vi "WriteCoreLoop_v2.vi"(5 "InitialFiles Format":T1=enum."Binary Files", 7 "Controls ref.":T2, 8 "data error in":errorcluster, 9 "data queue in":refnum<queue>, 10 "control queue in":errorcluster, 11 "control queue in":refnum<queue>) -> (0 "error out":errorcluster)   [LabVIEW 2013]
uses:
  ControlDef/Files_Format.ctl
  ControlDef/ProcessingMode.ctl
  Signal_Segment.ctl
  SaveControlsRef.ctl
  WriterState.ctl
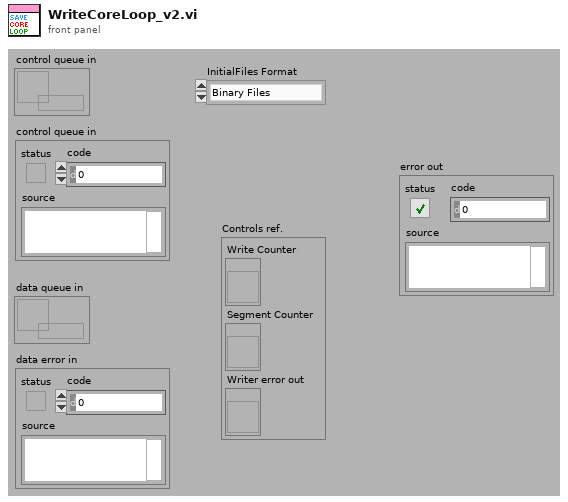
[diagram p1: front panel]
types:
  T1 = typedef "Files_Format.ctl" = enum16{"Text Files", "mzML Files", "Binary Files", "BioMap Files", "imzML Files"}
  T2 = typedef "SaveControlsRef.ctl" = cluster{"Write Counter":refnum<vi>, "Segment Counter":refnum<vi>, "Writer error out":refnum<vi>}
  T3 = typedef "WriterState.ctl" = cluster{"State":enum16{"Open", "Close", "ChangeFormat", "SetHeader", "QuitProg."}, "Params":variant}
  T4 = enum16{"Open", "Close", "ChangeFormat", "SetHeader", "QuitProg."}
  T5 = typedef "Signal_Segment.ctl" = cluster{"SampleRate":dbl, "TrigDelay":dbl, "SpecLength":dbl, "DAQ_Range":dbl, "Average#":i32, "Position":dbl[], "Spectrum":sgl[], "Calibr.":dbl[], "Pressure":dbl, "Desp_LaserEnergy":dbl, "PI_LaserEnergy":dbl, "Voltages Table":sgl[][], "ProcMode":T6, "Threshold":dbl, "Comment":string, "TickCount":dbl, "Time Stamp":timestamp}
  T6 = typedef "ProcessingMode.ctl" = enum16{"None", "Drop by Threshold", "TDC Simulate", "SetFilter"}
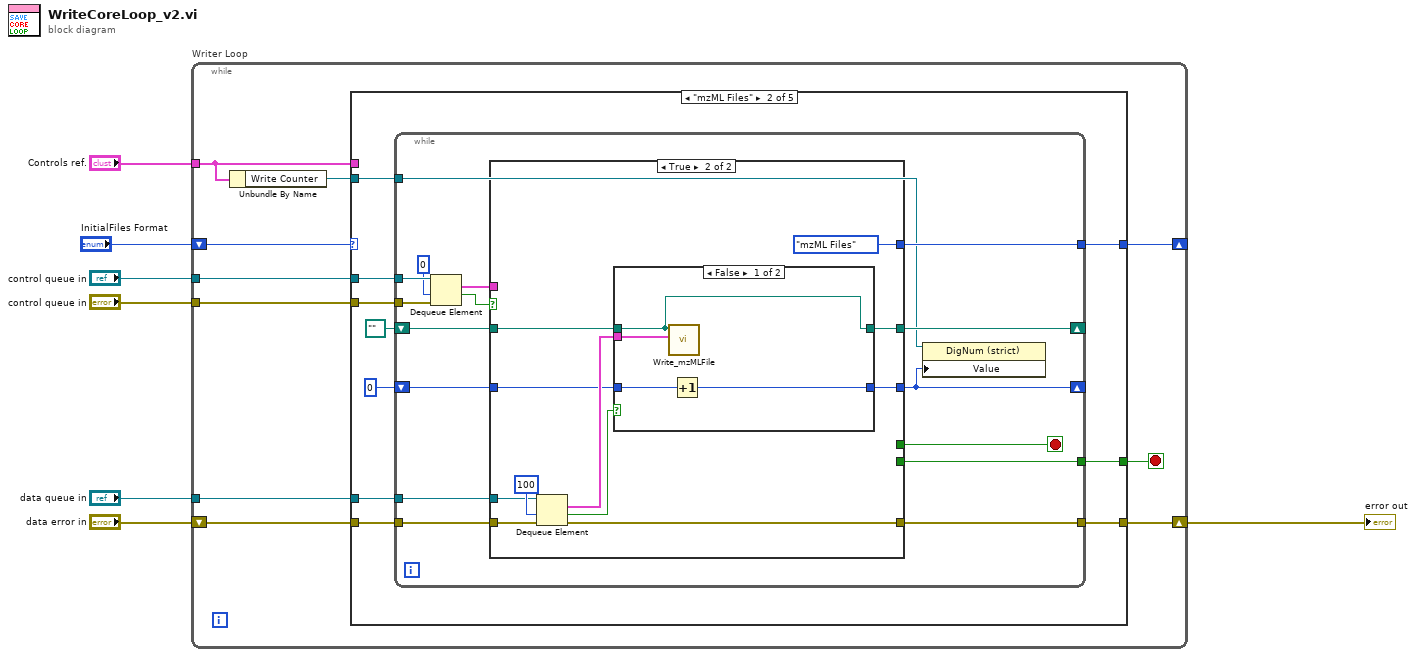
[diagram p0: block diagram]
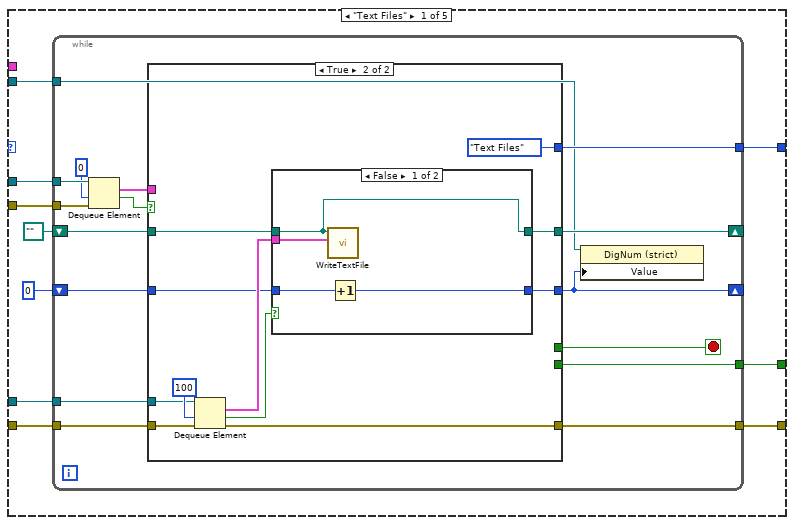
[diagram p2: hidden frame]
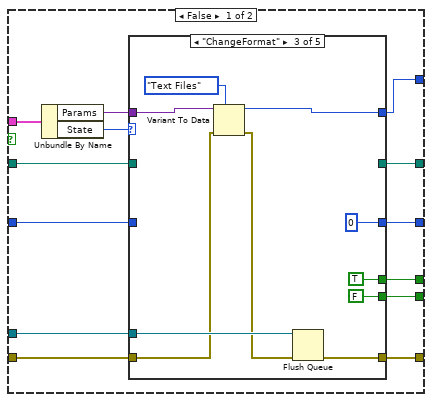
[diagram p3: hidden frame]
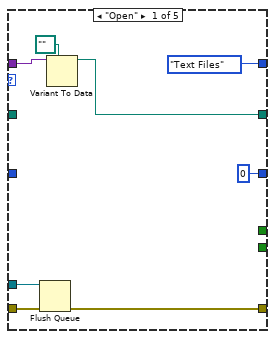
[diagram p4: hidden frame]
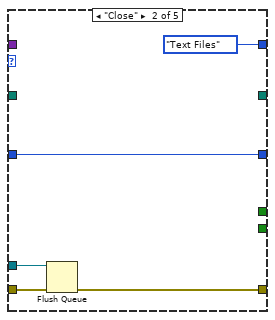
[diagram p5: hidden frame]
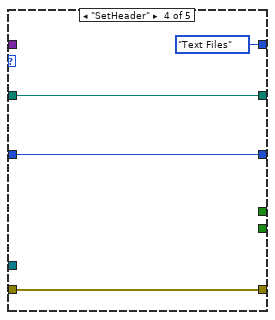
[diagram p6: hidden frame]
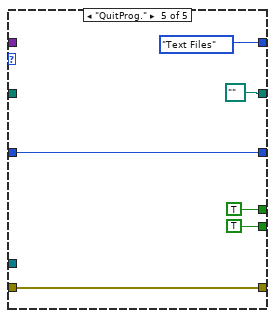
[diagram p7: hidden frame]
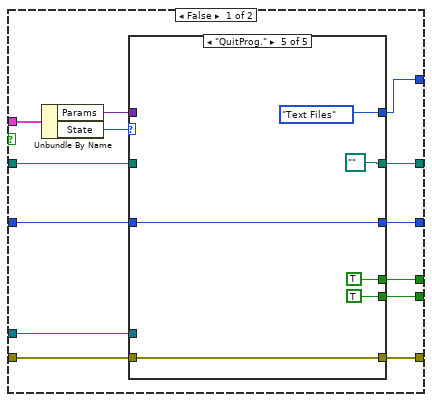
[diagram p9: hidden frame]
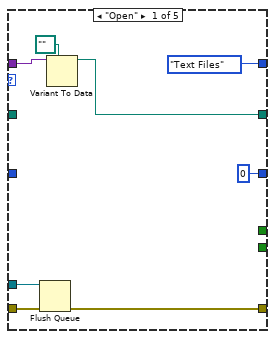
[diagram p10: hidden frame]
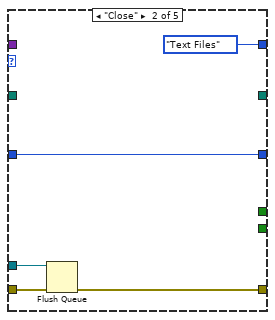
[diagram p11: hidden frame]
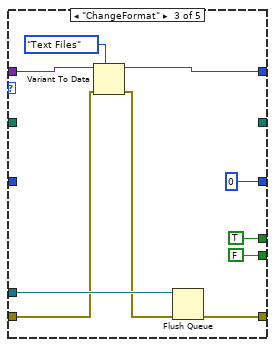
[diagram p12: hidden frame]
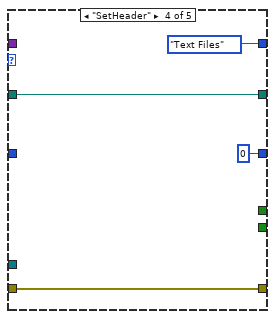
[diagram p13: hidden frame]
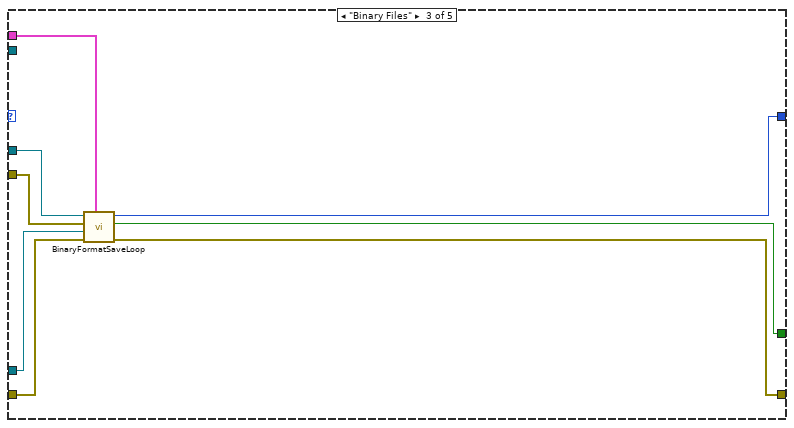
[diagram p15: hidden frame]
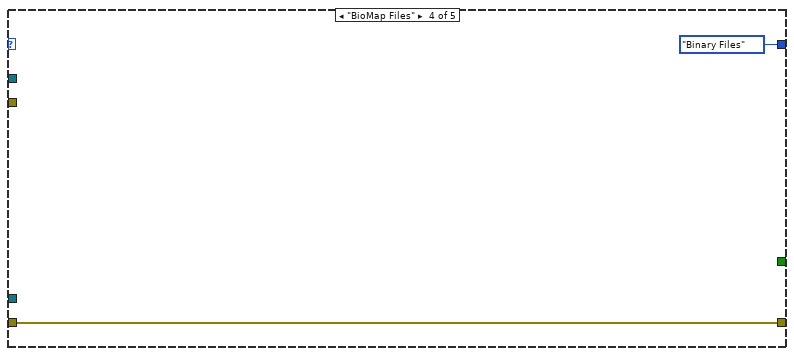
[diagram p16: hidden frame]
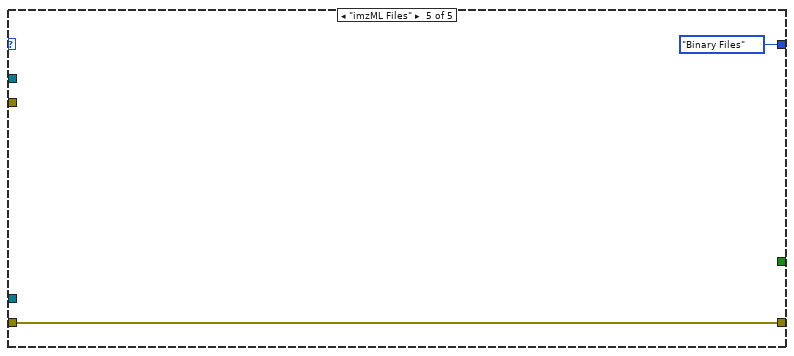
[diagram p17: hidden frame]
diagram:
  n1 = while "Writer Loop" {
    shift-right: [w10] -> w2
    shift-left: "data error in" -> [w15]
    tunnel: "data queue in" -> [w16]
    tunnel: "Controls ref." -> [w9]
    tunnel: "control queue in" -> [w14]
    tunnel: "control queue in" -> [w13]
    shift-right: [w11] -> _
    shift-left: "InitialFiles Format" -> [w12]
    stop <- w17 stop-if-true
    n2 = Unbundle By Name(w9) -> ("Write Counter"=w8:refnum<vi>)
    n3 = case shown="\"mzML Files\"" w12 {
      tunnel: [w27 w116 w203 _ _] -> w17
      tunnel: w16 -> [w25 w114 w202 _ _]
      tunnel: w15 -> [w24 w113 w201 w205 w207]
      tunnel: w14 -> [w23 w112 w200 _ _]
      tunnel: w13 -> [w22 w111 w199 _ _]
      tunnel: [w21 w110 w198 Files_Format."Binary Files" ("Format") Files_Format."Binary Files" ("Format")] -> w11
      tunnel: [w19 w108 w196 w205 w207] -> w10
      tunnel: w9 -> [_ _ w197 _ _]
      tunnel: w8 -> [w18 w107 _ _ _]
      frame "Text Files" {
        n4 = while {
          tunnel: [w41] -> w27
          shift-right: [w29] -> _
          shift-left: 0 -> [w43]
          tunnel: w25 -> [w36]
          tunnel: w24 -> [w35]
          shift-right: [w31] -> _
          shift-left: path "" ("file path") -> [w42]
          tunnel: w23 -> [w40]
          tunnel: w22 -> [w39]
          tunnel: [w32] -> w21
          tunnel: [w30] -> w19
          tunnel: w18 -> [w28]
          stop <- w33 stop-if-true
          n5 = Dequeue Element(queue=w40, timeout in ms (-1)=0, error in (no error)=w39) -> (element=w34:T3, timed out?=w37:bool)  [unwired: 2 out]
          n6 = case shown="True" w37 {
            tunnel: w43 -> [w50 w94]
            tunnel: w42 -> [w54 w96]
            tunnel: [w51 w93] -> w29
            tunnel: [w53 _] -> w41
            tunnel: w36 -> [w48 w99]
            tunnel: w35 -> [w47 w98]
            tunnel: w34 -> [w56 _]
            tunnel: [w52 _] -> w33
            tunnel: [w44 Files_Format."Text Files" ("Format")] -> w32
            tunnel: [w49 w91] -> w31
            tunnel: [w46 w90] -> w30
            frame False {
              n7 = Unbundle By Name(w56) -> ("Params"=w45:variant, "State"=w55:T4)
              n8 = case shown="\"ChangeFormat\"" w55 {
                tunnel: w54 -> [_ _ _ w81 _]
                tunnel: [w57 _ _ w81 path "" ("file path")] -> w49
                tunnel: [_ _ FALSE _ TRUE] -> w53
                tunnel: [_ _ TRUE _ TRUE] -> w52
                tunnel: [Files_Format."Text Files" ("Format") Files_Format."Text Files" ("Format") w73 Files_Format."Text Files" ("Format") Files_Format."Text Files" ("Format")] -> w44
                tunnel: [0 w69 0 w82 w87] -> w51
                tunnel: w50 -> [_ w69 _ w82 w87]
                tunnel: w48 -> [w61 w67 w76 _ _]
                tunnel: w47 -> [w62 w68 w71 w80 w84]
                tunnel: [w60 w66 w75 w80 w84] -> w46
                tunnel: w45 -> [w58 _ w74 _ _]
                frame "Open" {
                  n9 = Flush Queue(queue=w61, error in (no error)=w62) -> (error out=w60:errorcluster)  [unwired: 2 out]
                  n10 = Variant To Data(type=path "" ("path"), Variant=w58) -> (data=w57:path)  [unwired: 1 in, 1 out]
                }
                frame "Close" {
                  n11 = Flush Queue(queue=w67, error in (no error)=w68) -> (error out=w66:errorcluster)  [unwired: 2 out]
                }
                frame "ChangeFormat" {
                  n12 = Variant To Data(error in=w71, type=Files_Format."Text Files" ("Format"), Variant=w74) -> (data=w73:T1, error out=w72:errorcluster)
                  n13 = Flush Queue(queue=w76, error in (no error)=w72) -> (error out=w75:errorcluster)  [unwired: 2 out]
                }
                frame "SetHeader" {
                }
                frame "QuitProg." {
                }
              }
            }
            frame True {
              n14 = Dequeue Element(queue=w99, timeout in ms (-1)=100, error in (no error)=w98) -> (element=w97:T5, timed out?=w92:bool, error out=w90:errorcluster)  [unwired: 1 out]
              n15 = case shown="False" w92 {
                tunnel: w97 -> [w104 _]
                tunnel: w96 -> [w103 w106]
                tunnel: [w103 w106] -> w91
                tunnel: w94 -> [w102 w105]
                tunnel: [w101 w105] -> w93
                frame False {
                  n16 = call "WriteTextFile.vi"("Signal Segment"=w104, "Filename"=w103) -> ()  [unwired: 9 in, 1 out]
                  n17 = Increment(x=w102) -> (x+1=w101:i32)
                }
                frame True {
                }
              }
            }
          }
          n18 = property class="DigNum (strict)"(reference=w28, "Value"=w29) -> ()  [unwired: 1 in, 2 out]
        }
      }
      frame "mzML Files" {
        n19 = while {
          tunnel: [w130] -> w116
          shift-right: [w118] -> _
          shift-left: 0 -> [w132]
          tunnel: w114 -> [w125]
          tunnel: w113 -> [w124]
          shift-right: [w120] -> _
          shift-left: path "" ("file path") -> [w131]
          tunnel: w112 -> [w129]
          tunnel: w111 -> [w128]
          tunnel: [w121] -> w110
          tunnel: [w119] -> w108
          tunnel: w107 -> [w117]
          stop <- w122 stop-if-true
          n20 = Dequeue Element(queue=w129, timeout in ms (-1)=0, error in (no error)=w128) -> (element=w123:T3, timed out?=w126:bool)  [unwired: 2 out]
          n21 = case shown="True" w126 {
            tunnel: w132 -> [w139 w183]
            tunnel: w131 -> [w143 w185]
            tunnel: [w140 w182] -> w118
            tunnel: [w142 _] -> w130
            tunnel: w125 -> [w137 w188]
            tunnel: w124 -> [w136 w187]
            tunnel: w123 -> [w145 _]
            tunnel: [w141 _] -> w122
            tunnel: [w133 Files_Format."mzML Files" ("Format")] -> w121
            tunnel: [w138 w180] -> w120
            tunnel: [w135 w179] -> w119
            frame False {
              n22 = Unbundle By Name(w145) -> ("Params"=w134:variant, "State"=w144:T4)
              n23 = case shown="\"QuitProg.\"" w144 {
                tunnel: w143 -> [_ _ _ w170 _]
                tunnel: [w146 _ _ w170 path "" ("file path")] -> w138
                tunnel: [_ _ FALSE _ TRUE] -> w142
                tunnel: [_ _ TRUE _ TRUE] -> w141
                tunnel: [Files_Format."Text Files" ("Format") Files_Format."Text Files" ("Format") w162 Files_Format."Text Files" ("Format") Files_Format."Text Files" ("Format")] -> w133
                tunnel: [0 w158 0 0 w176] -> w140
                tunnel: w139 -> [_ w158 _ _ w176]
                tunnel: w137 -> [w150 w156 w165 _ _]
                tunnel: w136 -> [w151 w157 w160 w169 w175]
                tunnel: [w149 w155 w164 w169 w175] -> w135
                tunnel: w134 -> [w147 _ w163 _ _]
                frame "Open" {
                  n24 = Flush Queue(queue=w150, error in (no error)=w151) -> (error out=w149:errorcluster)  [unwired: 2 out]
                  n25 = Variant To Data(type=path "" ("path"), Variant=w147) -> (data=w146:path)  [unwired: 1 in, 1 out]
                }
                frame "Close" {
                  n26 = Flush Queue(queue=w156, error in (no error)=w157) -> (error out=w155:errorcluster)  [unwired: 2 out]
                }
                frame "ChangeFormat" {
                  n27 = Variant To Data(error in=w160, type=Files_Format."Text Files" ("Format"), Variant=w163) -> (data=w162:T1, error out=w161:errorcluster)
                  n28 = Flush Queue(queue=w165, error in (no error)=w161) -> (error out=w164:errorcluster)  [unwired: 2 out]
                }
                frame "SetHeader" {
                }
                frame "QuitProg." {
                }
              }
            }
            frame True {
              n29 = Dequeue Element(queue=w188, timeout in ms (-1)=100, error in (no error)=w187) -> (element=w186:T5, timed out?=w181:bool, error out=w179:errorcluster)  [unwired: 1 out]
              n30 = case shown="False" w181 {
                tunnel: w186 -> [w193 _]
                tunnel: w185 -> [w192 w195]
                tunnel: [w192 w195] -> w180
                tunnel: w183 -> [w191 w194]
                tunnel: [w190 w194] -> w182
                frame False {
                  n31 = call "Write_mzMLFile.vi"("Signal Segment"=w193, "Filename"=w192) -> ()  [unwired: 9 in, 1 out]
                  n32 = Increment(x=w191) -> (x+1=w190:i32)
                }
                frame True {
                }
              }
            }
          }
          n33 = property class="DigNum (strict)"(reference=w117, "Value"=w118) -> ()  [unwired: 1 in, 2 out]
        }
      }
      frame "Binary Files" {
        n34 = call "BinaryFormatSaveLoop.vi"("Controls ref."=w197, "data error in"=w201, "data queue in"=w202, 10:"control queue in"=w199, 11:"control queue in"=w200) -> ("queue error out"=w196:errorcluster, "Quit Binary"=w203:bool, "Format"=w198:T1)  [unwired: 3 in, 1 out]
      }
      frame "BioMap Files" {
      }
      frame "imzML Files" {
      }
    }
  }
  "error out" <- w2
